vi "PicoScope5000aExampleBlockMSO.vi"() -> ()   [LabVIEW 2010]
uses:
  shared/PicoBuffers.ctl
  <vilib>/Waveform/DWDTOps.llb/DWDT Analog to Digital.vi
  PicoScope5000aLib/PicoScope5000aAnalogChannelSettings.ctl
  PicoScope5000aLib/PicoScope5000aDigitalChannelSettings.ctl
  shared/Buffer and Transfer Settings.ctl
  shared/Acquisition Settings.ctl
panel:
  in  "Write to TDMS":bool
  in  "roundFaster":bool=TRUE
  in  "timeIntervalRequested":dbl min=0.0 format="%#6_6p"
  in  "Channel B Settings":T1={"Enabled"=FALSE, "Coupling"=1, "Range"=6, "Analogue Offset"=0.0, "Bandwidth Limit"=0} {"Bandwidth Limit" items=["Full", "20MHz"]; "Range" items=["10 mV", "20 mV", "50 mV", "100 mV", "200 mV", "500 mV", "1 V", "2 V", "5 V", "10 V", "20 V"]; "Coupling" items=["AC", "DC"]}
  out "overflow":i16 format="%010b"
  in  "Apply Settings":bool
  in  "Port 0 Settings":T2={"Enabled"=FALSE, "Logic Level"=9830} {"Logic Level" items=["1.5V TTL"=9830, "2.5V CMOS"=16383]}
  in  "Channel A Settings":T1={"Enabled"=TRUE, "Coupling"=1, "Range"=6, "Analogue Offset"=0.0, "Bandwidth Limit"=0} {"Bandwidth Limit" items=["Full", "20MHz"]; "Range" items=["10 mV", "20 mV", "50 mV", "100 mV", "200 mV", "500 mV", "1 V", "2 V", "5 V", "10 V", "20 V"]; "Coupling" items=["AC", "DC"]}
  in  "Trigger Settings":T3={"Trigger Enabled"=FALSE, "Trigger Source"=enum."Channel A", "Trigger Threshold (volts)"=0.0, "Trigger Direction"=2, "Trigger Delay (samples)"=0, "Auto Trigger Time (ms)"=1000} {"Trigger Direction" items=["Rising"=2, "Falling"=3]}
  out "USB 3.0 device on non-USB 3.0 Port":bool=TRUE
  out "USB Powered":bool=TRUE
  out "Device Info":T4={"Driver Version"="2.1.104.3324", "USB Version"="2.0", "Hardware"="1", "Variant"="5244A", "Batch and Serial"="CQ178/007", "Cal Date"="11Jun13", "Kernel Version"="1.0", "Digital HW Version"="1", "Analogue HW Version"="1", "MSO"=FALSE, "Number of channels"=2}
  out "error out":errorcluster
  in  "Data file":path=path "PicoScope5000aExampleBlock Data"
  in  "Buffer and Transfer Settings":T5={"startIndex"=0, "Samples"=1000000, "Down Sample Ratio"=1, "Down-Sample Mode"=0} {"Down-Sample Mode" items=["RAW none"=2147483648, "None"=0, "Aggregate"=1, "Decimate"=2, "Average"=4]; "Down Sample Ratio" step=1; "Samples" format="%_6p"}
  in  "Acquisition Settings":T6={"preTriggerSamples"=0, "postTriggerSamples"=1000000, "timebase"=0} {"postTriggerSamples" format="%_6p"; "preTriggerSamples" format="%_6p"}
  out "Properties Panel":T7={"Sample Frequency"=41666668.0, "Sample Rate"=2.4000000209412065e-08, "Max Samples Available"=26843008, "Number of Samples"=0, "Total Capture Time (sec) "=0.0, "Max Total Capture Time Available (sec)"=0.6442322134971619} {"Max Total Capture Time Available (sec)" format="%.3p"; "Sample Frequency" format="%.6p"; "Sample Rate" format="%.3p"; "Max Samples Available" format="%_6p"; "Total Capture Time (sec)" format="%.3p"}
  out "Port 0":digitalwaveform(graph)={"t0"=timestamp(0 s since 1904-01-01), "dt"=8e-09, "Y"={"transitions"=[], "data"=[]}}
  in  "stop":bool
  out "Analog Channels":cluster{i32, sgl, "Data":dbl[]}[](graph)
  in  "Resolution":u32(ring) items=["8-bit"=0, "12-bit"=1, "14-bit"=2, "15-bit"=3, "16-bit"=4, "10-bit"=10]
  in  "Serial Number":string
  in  "Use Serial Number":bool
  in  "error in (no error)":errorcluster
  # "Bit 0 = ChA"
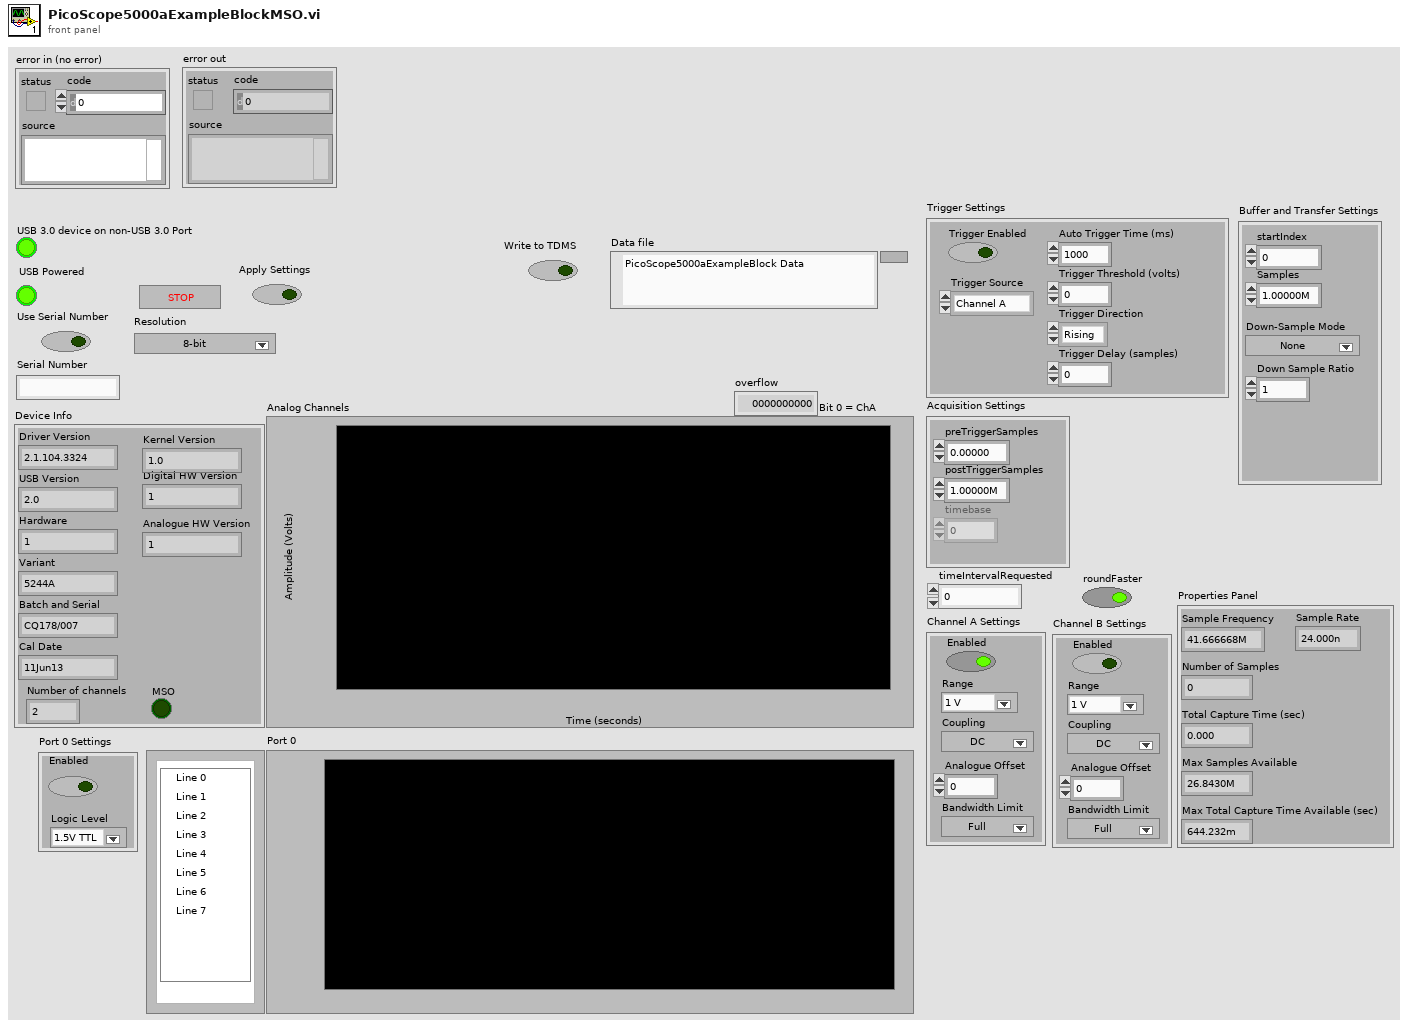
[diagram p1: front panel]
types:
  T1 = typedef "PicoScope5000aAnalogChannelSettings.ctl" = cluster{"Enabled":bool, "Coupling":i16, "Range":u16, "Analogue Offset":sgl, "Bandwidth Limit":u32}
  T2 = typedef "PicoScope5000aDigitalChannelSettings.ctl" = cluster{"Enabled":bool, "Logic Level":i16}
  T3 = cluster{"Trigger Enabled":bool, "Trigger Source":enum16{"Channel A", "Channel B", "Channel C", "Channel D", "Ext."}, "Trigger Threshold (volts)":dbl, "Trigger Direction":u16, "Trigger Delay (samples)":u32, "Auto Trigger Time (ms)":i16}
  T4 = cluster{"Driver Version":string, "USB Version":string, "Hardware":string, "Variant":string, "Batch and Serial":string, "Cal Date":string, "Kernel Version":string, "Digital HW Version":string, "Analogue HW Version":string, "MSO":bool, "Number of channels":i16}
  T5 = typedef "Buffer and Transfer Settings.ctl" = cluster{"startIndex":u64, "Samples":u64, "Down Sample Ratio":u64, "Down-Sample Mode":u32}
  T6 = typedef "Acquisition Settings.ctl" = cluster{"preTriggerSamples":u64, "postTriggerSamples":u64, "timebase":u32}
  T7 = cluster{"Sample Frequency":dbl, "Sample Rate":dbl, "Max Samples Available":u64, "Number of Samples":u64, "Total Capture Time (sec) ":dbl, "Max Total Capture Time Available (sec)":dbl}
  T8 = typedef "PicoBuffers.ctl" = cluster{"Max Buffer Pointers":u64[][][], "Min Buffer Pointers":u64[][][], "StreamingDataInfo":cluster{"Channel":u32, "Down-Sample Mode":u32, "PICO_DATA_TYPE":enum32{"PICO_INT8_T", "PICO_INT16_T", "PICO_INT32_T", "PICO_UINT32_T", "PICO_INT64_T", ""}, "Samples":i32, "bufferIndex":u64, "startIndex":i32, "overflow":i16}[][]}
  T9 = enum16{"open", "open or create", "create or replace", "create", "open (read-only)"}
  T10 = cluster{"Sample Frequency":sgl, "Sample Rate":sgl, "Max Samples Available":i32, "Number of Samples":u32, "Total Capture Time (sec) ":sgl, "Max Total Capture Time Available (sec)":sgl}
  T11 = cluster{"Channel A Buffer":i16[], "Channel B Buffer":i16[], "Channel C Buffer":i16[], "Channel D Buffer":i16[], "Channel E Buffer":i16[], "Channel F Buffer":i16[], "Channel G Buffer":i16[], "Channel H Buffer":i16[], "Port 0 Buffer":i16[], "Port 1 Buffer":i16[]}[]
  T12 = cluster{"Channel A Buffer":i16[], "Channel B Buffer":i16[], "Channel C Buffer":i16[], "Channel D Buffer":i16[], "Channel E Buffer":i16[], "Channel F Buffer":i16[], "Channel G Buffer":i16[], "Channel H Buffer":i16[], "Port 0 Buffer":i16[], "Port 1 Buffer":i16[]}
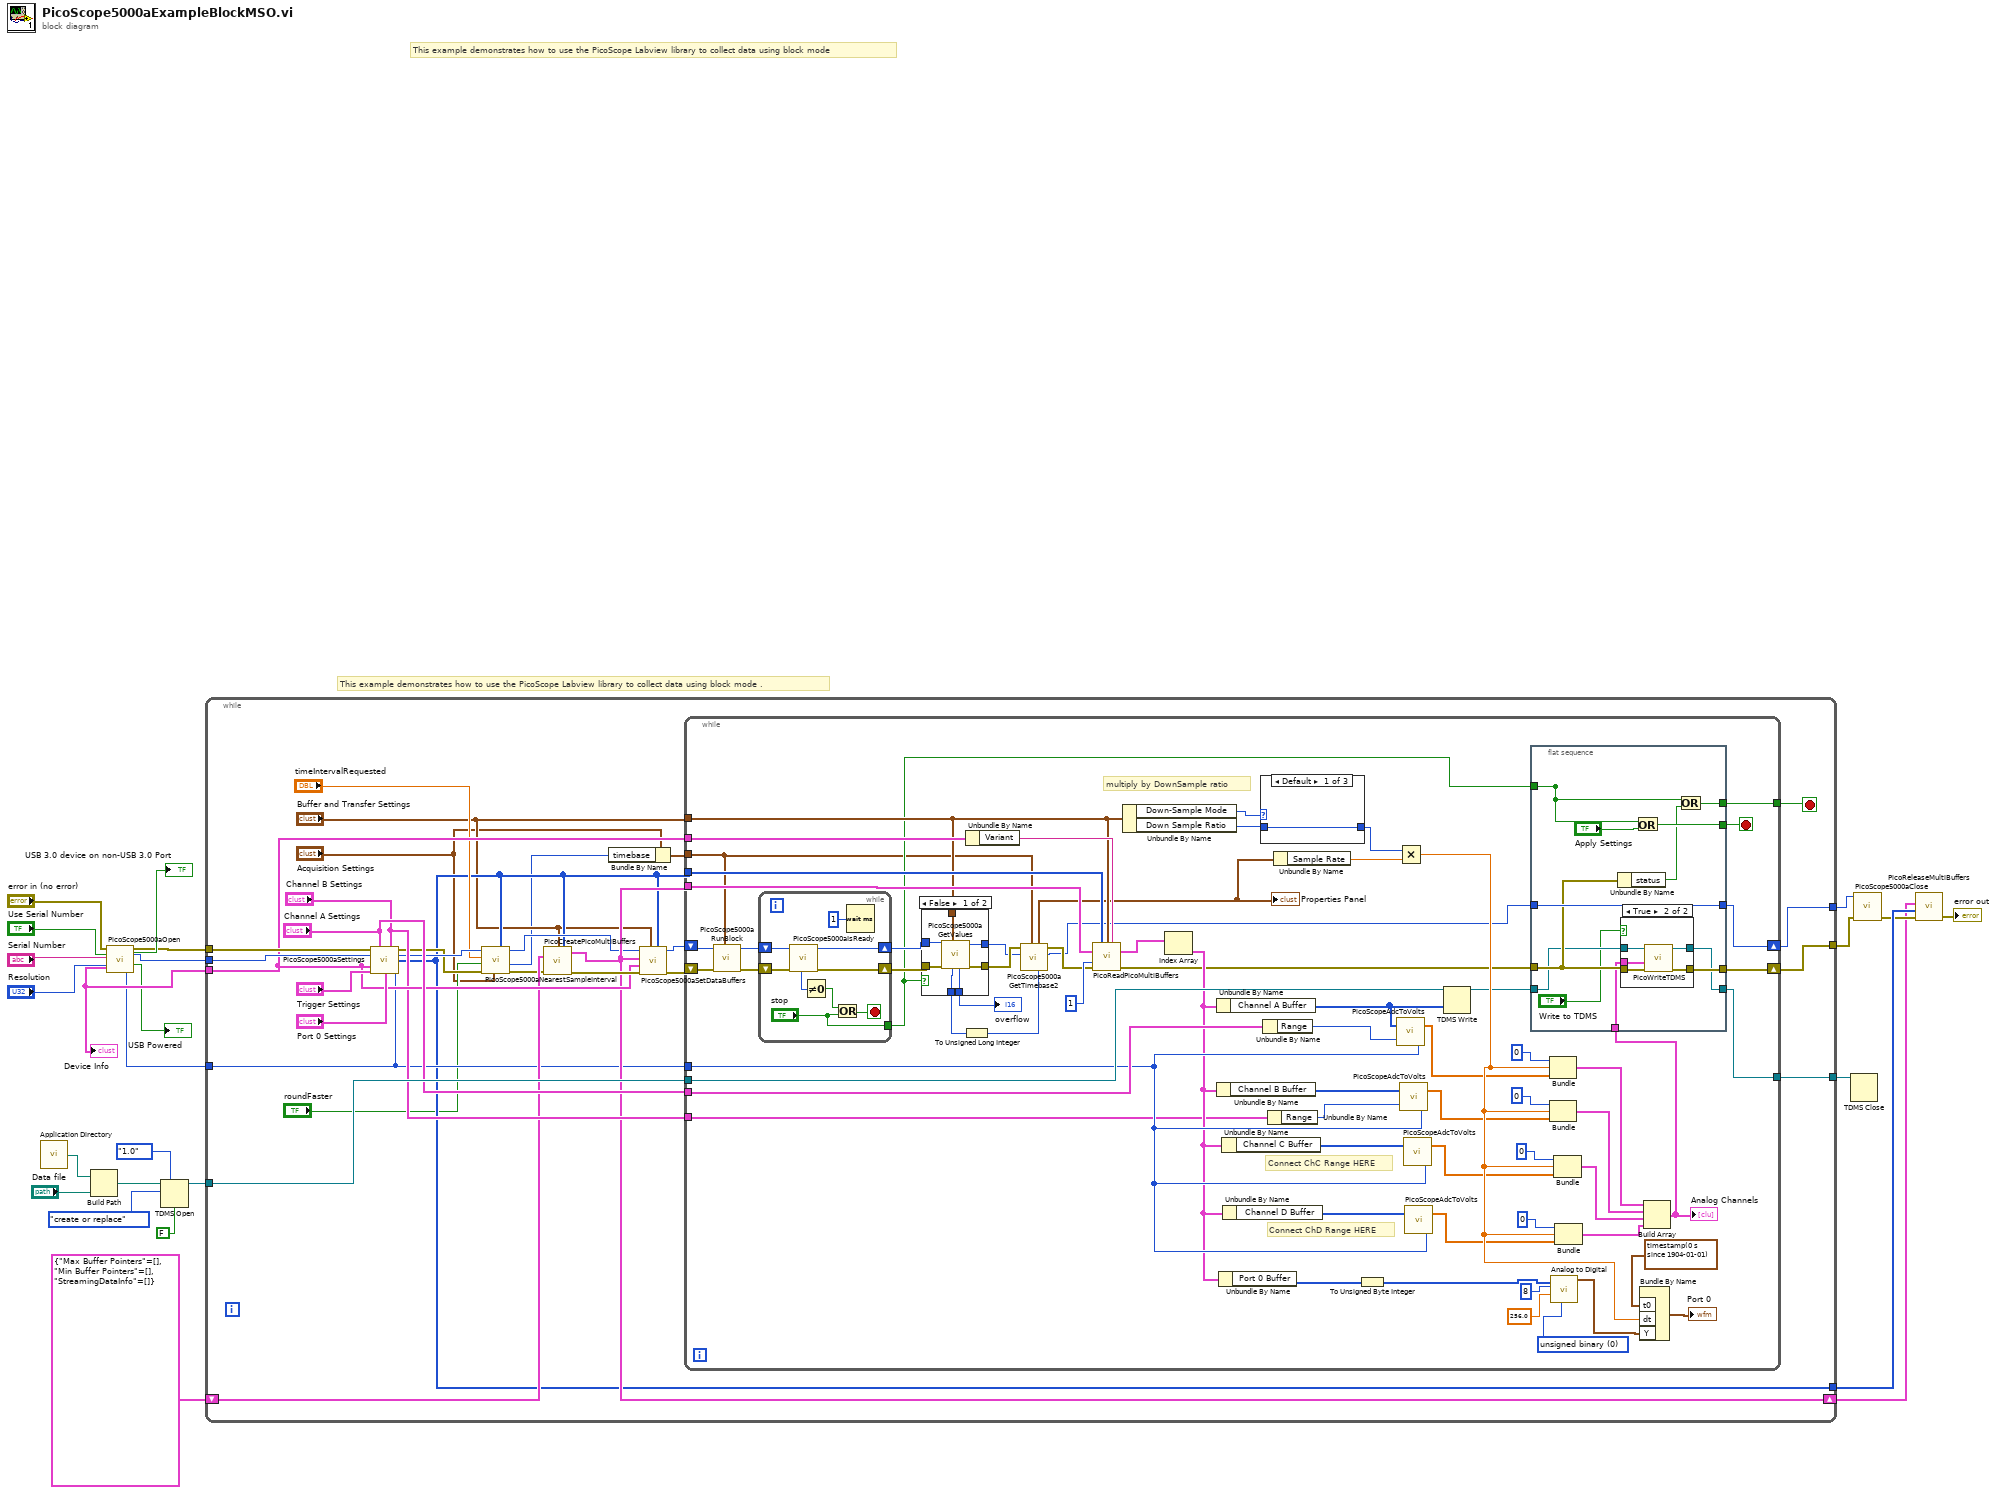
[diagram p0: block diagram]
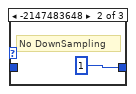
[diagram p4: hidden frame]
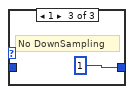
[diagram p5: hidden frame]
diagram:
  # "This example demonstrates how to use the PicoScope Labview library to collect data using block mode ."
  # "This example demonstrates how to use the PicoScope Labview library to collect data using block mode"
  n1 = call <vilib>:"Application Directory.vi"() -> ("Application Directory"=w18:path)
  n2 = Build Path(base path=w18, name or relative path="Data file") -> (appended path=w19:path)
  n3 = call "PicoScope5000aOpen.vi"("error in (no error)"="error in (no error)", "Serial Number"="Serial Number", "Use Serial Number"="Use Serial Number", "Resolution"="Resolution") -> ("USB 3.0 device on non-USB 3.0 Port"=→"USB 3.0 device on non-USB 3.0 Port":bool, "error out"=w6:errorcluster, "handle"=w25:i16, "USB Powered"=→"USB Powered":bool, "Device Info"=w10:T4, "Max ADC value"=w9:i16)  [unwired: 6 in]
  "Device Info" <- w10
  n4 = TDMS Open(6:FALSE ("disable buffering? (T)"), 7:enum16{"1.0", "2.0"}."1.0" ("file format version (2.0)"), 10:T9."create or replace" ("operation (0:open)"), 11:w19) -> (3:w16:refnum<k34>)  [unwired: 2 in, 1 out]
  n5 = while {
    tunnel: w25 -> [w52]
    tunnel: w9 -> [w35]
    tunnel: [w31] -> w24
    tunnel: [w46] -> w17
    tunnel: w16 -> [w53]
    tunnel: w10 -> [w41]
    tunnel: w6 -> [w51]
    tunnel: [w47] -> w4
    tunnel: [w44] -> w5
    shift-right: [w38] -> w1
    shift-left: T8 {"Max Buffer Pointers"=[], "Min Buffer Pointers"=[], "StreamingDataInfo"=[]} ("Data Pointers") -> [w39]
    stop <- w45 stop-if-true
    n6 = call "PicoScope5000aSettings.vi"("error in"=w51, "Channel A Settings"="Channel A Settings", "Port 0 Settings"="Port 0 Settings", "Channel B Settings"="Channel B Settings", "handle in"=w52, "Device Info"=w41, "Trigger Settings"="Trigger Settings", "Max ADC value"=w35) -> ("error out"=w34:errorcluster, "handle out"=w36:i16, "enabled array"=w31:i16[])  [unwired: 5 in]
    n7 = call "PicoScope5000aNearestSampleInterval.vi"("Enabled array"=w31, "Acquisition Settings"="Acquisition Settings", "error in (no error)"=w34, "roundFaster"="roundFaster", "timeIntervalRequested"="timeIntervalRequested", "handle in"=w36) -> ("error out"=w37:errorcluster, "timebase"=w26:u32, "handle out"=w33:i16)  [unwired: 2 in, 1 out]
    n8 = call "PicoCreatePicoMultiBuffers.vi"("Buffer and Transfer Settings"="Buffer and Transfer Settings", "enabled array"=w31, "Data Pointers In"=w39, "error in (no error)"=w37) -> ("Data Pointers"=w38:T8, "error out"=w54:errorcluster)  [unwired: 10 in]
    n9 = Bundle By Name(cluster="Acquisition Settings", "timebase"=w26) -> (w28:T6)
    n10 = call "PicoScope5000aSetDataBuffers.vi"("enabled array"=w31, "Buffer and Transfer Settings"="Buffer and Transfer Settings", "error in (no error)"=w54, "Device Info"=w41, "Data Pointers In"=w38, "handle in"=w33) -> ("error out"=w43:errorcluster, "handle out"=w42:i16)  [unwired: 4 in]
    n11 = while {
      tunnel: w38 -> [w121]
      tunnel: "Buffer and Transfer Settings" -> [w70]
      tunnel: w31 -> [w112]
      tunnel: "Channel A Settings" -> [w111]
      tunnel: w28 -> [w62]
      tunnel: w35 -> [w110]
      tunnel: w41 -> [w107]
      tunnel: [w77] -> w45
      shift-right: [w81] -> w47
      shift-left: w43 -> [w71]
      shift-right: [w75] -> w44
      shift-left: w42 -> [w72]
      tunnel: w53 -> [w120]
      tunnel: [w79] -> w46
      tunnel: "Channel B Settings" -> [w58]
      stop <- w76 stop-if-true
      w97 = u16 0 items=["unsigned binary", "offset binary", "2's complement"] ("data format (offset binary)")
      # "Connect ChD Range HERE"
      # "Connect ChC Range HERE"
      # "multiply by DownSample ratio"
      n12 = call "PicoScope5000aRunBlock.vi"("Acquisition Settings"=w62, "error in (no error)"=w71, "handle in"=w72) -> ("error out"=w114:errorcluster, "handle out"=w113:i16)  [unwired: 5 in, 2 out]
      n13 = while {
        shift-right: [w157] -> w73
        shift-left: w114 -> [w158]
        shift-right: [w156] -> w74
        shift-left: w113 -> [w155]
        tunnel: ["stop"] -> w69
        stop <- w152 stop-if-true
        n14 = call "PicoScope5000aIsReady.vi"("error in (no error)"=w158, "handle in"=w155) -> ("error out"=w157:errorcluster, "handle out"=w156:i16, "ready"=w154:i16)  [unwired: 7 in]
        n15 = Not Equal To 0?(x=w154) -> (x != 0?=w153:bool)
        n16 = Or(x=w153, y="stop") -> (x .or. y?=w152:bool)
        n17 = Wait (ms)(milliseconds to wait=u32 1) -> ()  [unwired: 1 out]
      }
      n18 = case shown="False" w69 {
        tunnel: w73 -> [w128 w129]
        tunnel: w74 -> [w127 w130]
        tunnel: [w126 w130] -> w66
        tunnel: [w125 w129] -> w67
        tunnel: w70 -> [w124 _]
        tunnel: [w123 _] -> w68
        tunnel: [w122 _] -> w61
        frame False {
          n19 = call "PicoScope5000aGetValues.vi"("Buffer and Transfer Settings"=w124, "error in (no error)"=w128, "handle in"=w127) -> ("error out"=w125:errorcluster, "handle out"=w126:i16, "overflow"=w123:i16, "noOfSamples"=w122:u64)  [unwired: 5 in]
        }
        frame True {
        }
      }
      "overflow" <- w68
      n20 = To Unsigned Long Integer(number=w61) -> (unsigned 32bit integer=w60:u32)
      n21 = Unbundle By Name(w107) -> ("Variant"=w108:string)
      n22 = call "PicoScope5000aGetTimebase2.vi"("Number of Samples"=w60, "Acquisition Settings"=w62, "handle in"=w66, "error in (no error)"=w67) -> ("handle out"=w64:i16, "error out"=w65:errorcluster, "Properties Panel"=w63:T10)  [unwired: 5 in]
      "Properties Panel" <- w63
      n23 = call "PicoReadPicoMultiBuffers.vi"("enabled array"=w112, "Buffer and Transfer Settings"=w70, "Variant"=w108, "Data Pointers"=w121, "No of Buffers"=1, "error in (no error)"=w65) -> ("MultiBuffers (Max or non-aggregated)"=w119:T11, "error out"=w78:errorcluster)  [unwired: 7 in, 1 out]
      n24 = Unbundle By Name(w70) -> ("Down-Sample Mode"=w117:u32, "Down Sample Ratio"=w118:u64)
      n25 = Index Array(array=w119) -> (element=w82:T12)  [unwired: 1 in]
      n26 = Unbundle By Name(w82) -> ("Channel A Buffer"=w91:i16[])
      n27 = Unbundle By Name(w82) -> ("Channel B Buffer"=w102:i16[])
      n28 = Unbundle By Name(w82) -> ("Port 0 Buffer"=w56:i16[])
      n29 = Unbundle By Name(w82) -> ("Channel C Buffer"=w89:i16[])
      n30 = Unbundle By Name(w82) -> ("Channel D Buffer"=w85:i16[])
      n31 = case shown="Default" w117 {
        tunnel: [w159 u64 1 ("Down Sample Ratio") u64 1 ("Down Sample Ratio")] -> w115
        tunnel: w118 -> [w159 _ _]
        frame Default {
        }
        frame -2147483648 {
          # "No DownSampling"
        }
        frame 1 {
          # "No DownSampling"
        }
      }
      n32 = Unbundle By Name(w111) -> ("Range"=w104:u16)
      n33 = Unbundle By Name(w58) -> ("Range"=w59:u16)
      n34 = Unbundle By Name(w63) -> ("Sample Rate"=w109:sgl)
      n35 = To Unsigned Byte Integer(number=w56) -> (unsigned 8bit integer=w55:u8[])
      n36 = call "PicoScopeAdcToVolts.vi"("Max_adc"=w110, "Range Index"=w104, "Data"=w91) -> ("Data"=w92:dbl[])
      n37 = Multiply(x=w115, y=w109) -> (x*y=w116:sgl)
      n38 = call "PicoScopeAdcToVolts.vi"("Max_adc"=w110, "Range Index"=w59, "Data"=w102) -> ("Data"=w101:dbl[])
      n39 = call "PicoScopeAdcToVolts.vi"("Max_adc"=w110, "Data"=w89) -> ("Data"=w88:dbl[])  [unwired: 1 in]
      n40 = call "PicoScopeAdcToVolts.vi"("Max_adc"=w110, "Data"=w85) -> ("Data"=w84:dbl[])  [unwired: 1 in]
      n41 = TDMS Write(0:w120, 9:w91) -> (4:w80:refnum<k34>)  [unwired: 4 in, 3 out]
      n42 = flat-sequence {
        tunnel: [w142] -> w76
        tunnel: [w137] -> _
        tunnel: [w139] -> w77
        tunnel: w64 -> [w138]
        tunnel: [w138] -> w75
        tunnel: w78 -> [w135]
        tunnel: [w136] -> w81
        tunnel: [w134] -> w79
        tunnel: w80 -> [w133]
        tunnel: w69 -> [w137]
        tunnel: w57 -> [w131]
        frame #0 {
          n43 = Unbundle By Name(w135) -> ("status"=w140:bool)
          n44 = case shown="True" "Write to TDMS" {
            tunnel: w135 -> [w143 w149]
            tunnel: [w143 w148] -> w136
            tunnel: w133 -> [w144 w147]
            tunnel: [w144 w146] -> w134
            tunnel: w131 -> [_ w145]
            frame False {
            }
            frame True {
              n45 = call "PicoWriteTDMS.vi"("error in (no error)"=w149, "Analog Channels"=w145, "Refnum in"=w147) -> ("error out"=w148:errorcluster, "Refnum out"=w146:refnum<k34>)  [unwired: 7 in]
            }
          }
          n46 = Or(x=w137, y="Apply Settings") -> (x .or. y?=w142:bool)
          n47 = Or(x=w137, y=w140) -> (x .or. y?=w139:bool)
        }
      }
      n48 = Bundle(0, w116, "Data"=w92) -> (w100:cluster{i32, sgl, "Data":dbl[]})  [unwired: 1 in]
      n49 = Bundle(0, w116, "Data"=w101) -> (w99:cluster{i32, sgl, "Data":dbl[]})  [unwired: 1 in]
      n50 = call-poly <vilib>:"Analog to Digital.vi"("data format (offset binary)"=w97, "full-scale range (pk-pk)"=256.0, "resolution (16 bit)"=8, "analog waveform"=w55) -> ("digital waveform"=w93:digitalwaveform)  [unwired: 4 in, 3 out]
      n51 = Bundle(0, w116, "Data"=w88) -> (w87:cluster{i32, sgl, "Data":dbl[]})  [unwired: 1 in]
      n52 = Bundle(0, w116, "Data"=w84) -> (w83:cluster{i32, sgl, "Data":dbl[]})  [unwired: 1 in]
      n53 = Bundle By Name("t0"=timestamp(0 s since 1904-01-01), "dt"=w116, "Y"=w93) -> (→"Port 0":digitalwaveform)  [unwired: 1 in]
      n54 = Build Array(w100, w99, w87, w83) -> (w57:cluster{i32, sgl, "Data":dbl[]}[])
      "Analog Channels" <- w57
    }
  }
  n55 = TDMS Close(11:w17) -> ()  [unwired: 1 in, 2 out]
  n56 = call "PicoScope5000aClose.vi"("error in (no error)"=w4, "handle in"=w5) -> ("error out"=w3:errorcluster)  [unwired: 8 in, 1 out]
  n57 = call "PicoReleaseMultiBuffers.vi"("error in (no error)"=w3, "Enabled array"=w24, "Data Pointers"=w1) -> ("error out"=→"error out":errorcluster)  [unwired: 7 in, 1 out]
